vi "Configure.vi"(7 "Stopped Notification":refnum<notifier>, 8 "error in":errorcluster, 9 "Processed Display":refnum<vi>, 10 "Count Display":refnum<vi>, 11 "Actor in":refnum<class "CounterActor.lvclass">) -> (0 "error out":errorcluster, 3 "Actor out":refnum<class "CounterActor.lvclass">)   [LabVIEW 2026, in "CounterActor.lvclass"]
doc: "Message Counter actor method: Configure. Counter and Processed are private actor state."
uses:
  CounterActor.lvclass
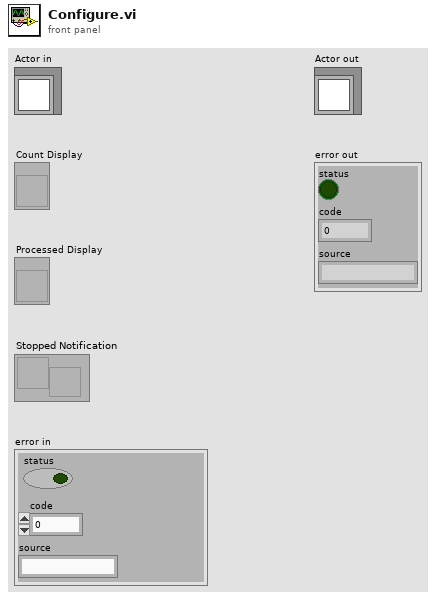
[diagram p1: front panel]
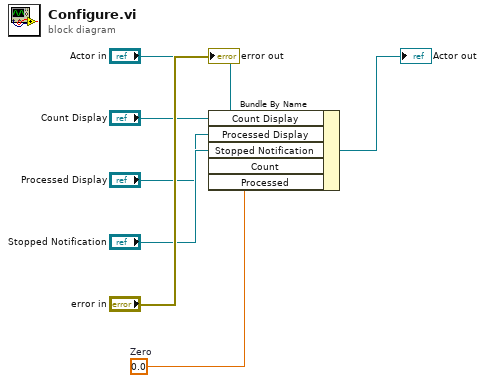
[diagram p0: block diagram]
diagram:
  w6 = 0.0  # Zero
  n1 = Bundle By Name(cluster="Actor in", "Count Display"="Count Display", "Processed Display"="Processed Display", "Stopped Notification"="Stopped Notification", "Count"=w6, "Processed"=w6) -> (→"Actor out":refnum<class "CounterActor.lvclass">)
  "error out" <- "error in"
